vi "SPARK Get Power Config.vi"   [LabVIEW 2027]
doc: "Get the power configuration of the SPARK."
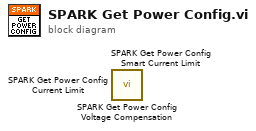
[diagram p0: block diagram]
diagram:
  n1 = call <vilib>:"SPARK Get Power Config Voltage Compensation.vi"() -> ()  [unwired: 8 in, 4 out]
  n2 = call <vilib>:"SPARK Get Power Config Smart Current Limit.vi"() -> ()  [unwired: 7 in, 5 out]
  n3 = call <vilib>:"SPARK Get Power Config Current Limit.vi"() -> ()  [unwired: 8 in, 4 out]
